vi "detect network devices.vi"(4 "remote timeout (300,000 ms)":u32=300000, 6 "detect all (F)":bool, 7 "local subnet only (F)":bool, 8 "error in":errorcluster, 10 "device class":T2, 11 "system session (localhost)":refnum<k21>="localhost") -> (0 "error out":errorcluster, 2 "devices":T1[](array[typedef]) {"product ID" format="%.0x"}, 3 "system session out":refnum<k21>)   [LabVIEW 2014, in "SMI.lvlib" / "Device.lvclass"]
uses:
  Device.lvclass
  device class selection.ctl
  network device information.ctl
  <vilib>/nisyscfg/Filter Mode.ctl
  <vilib>/nisyscfg/Close (Filter).vi
  <vilib>/nisyscfg/Close (Resources).vi
  <vilib>/regexp/Match Regular Expression.xnode
  <vilib>/nisyscfg/nisyscfg.lvlib
  <resource>/objmgr/niflexriosae.rc
  SMI.lvlib
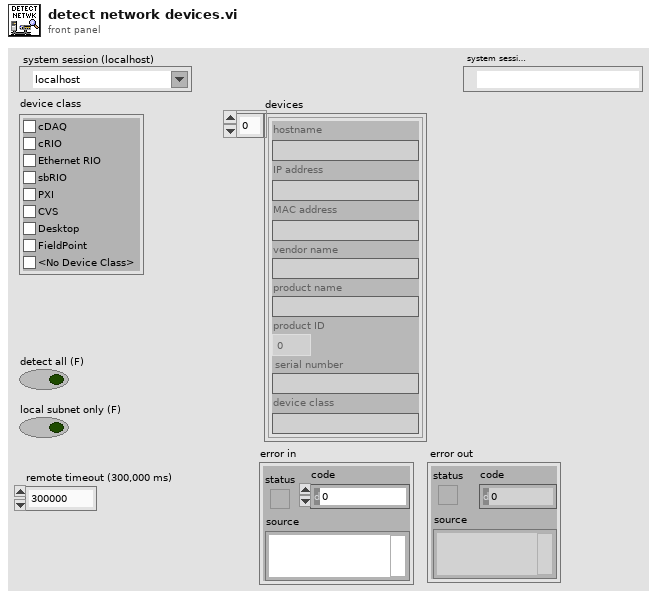
[diagram p1: front panel]
types:
  T1 = typedef "SMI.lvlib/Device.lvclass/network device information.ctl" = cluster{"hostname":string, "IP address":string, "MAC address":string, "vendor name":string, "product name":string, "product ID":u16, "serial number":string, "device class":string}
  T2 = typedef "SMI.lvlib/Device.lvclass/device class selection.ctl" = cluster{"cDAQ":bool, "cRIO":bool, "Ethernet RIO":bool, "sbRIO":bool, "PXI":bool, "CVS":bool, "Desktop":bool, "FieldPoint":bool, "<No Device Class>":bool}
  T3 = typedef "nisyscfg.lvlib/Filter Mode.ctl" = i32
  T4 = typedef "SMI.lvlib/Device.lvclass/device class.ctl" = enum16{"cDAQ", "cRIO", "Ethernet RIO", "sbRIO", "PXI", "CVS", "Desktop", "FieldPoint", "<No Device Class>", "<Detect All>"}
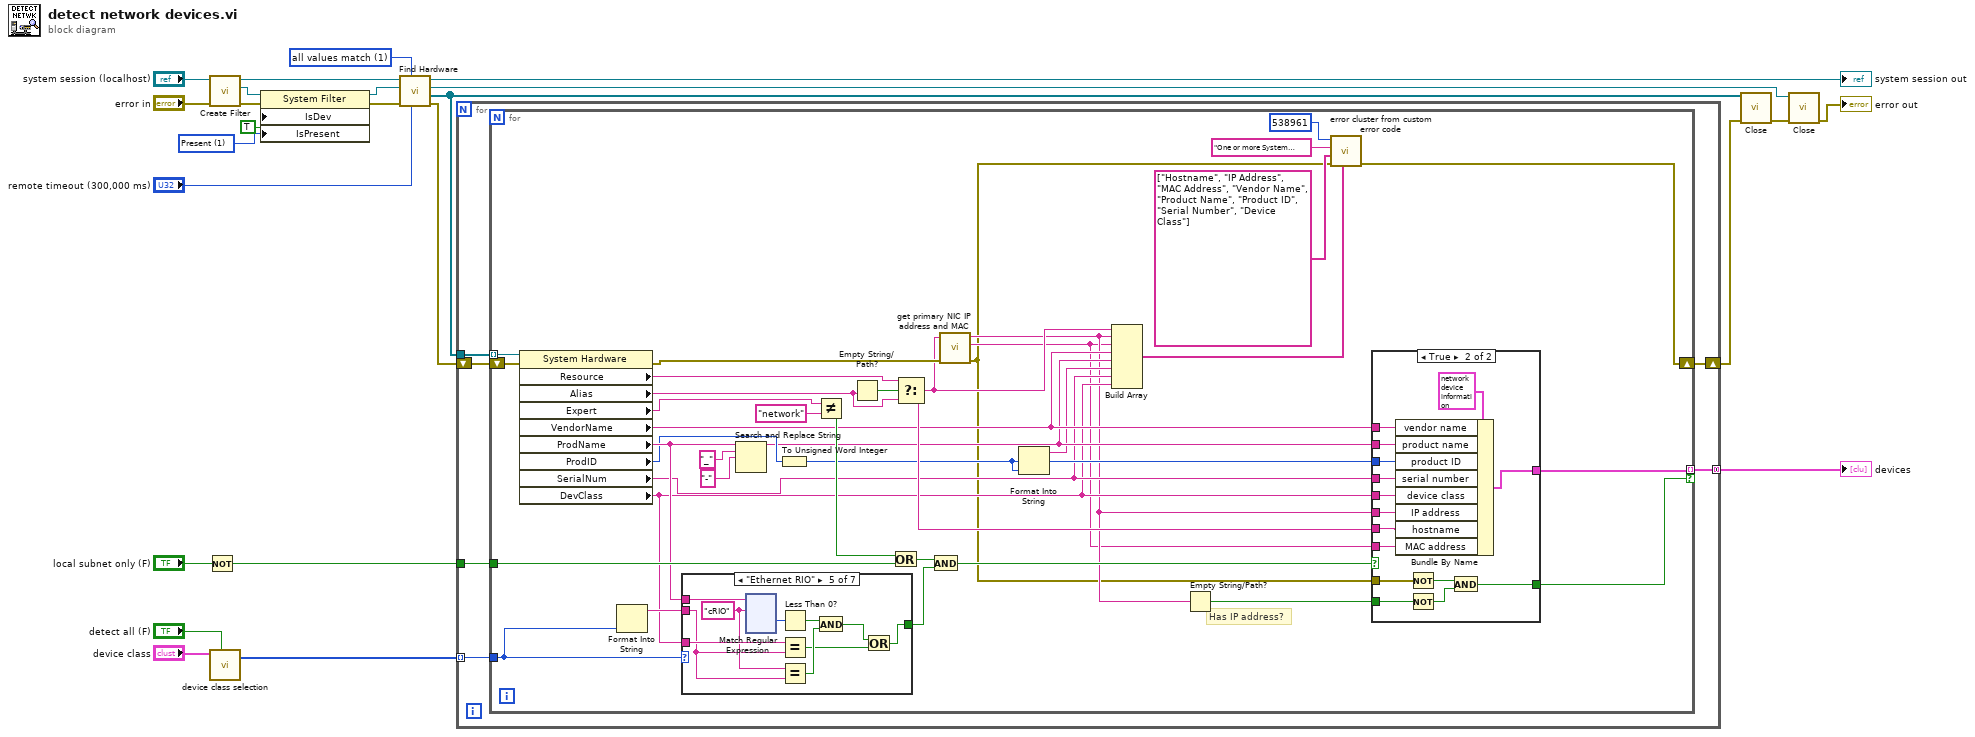
[diagram p0: block diagram]
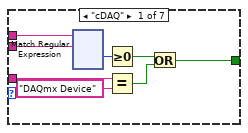
[diagram p3: hidden frame]
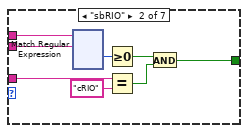
[diagram p4: hidden frame]
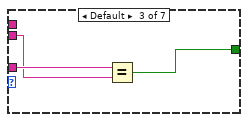
[diagram p5: hidden frame]
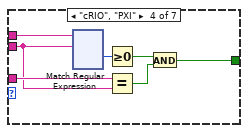
[diagram p6: hidden frame]
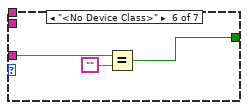
[diagram p7: hidden frame]
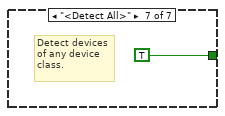
[diagram p8: hidden frame]
diagram:
  w4 = 1 items=["Initializing"=-2, "Unknown"=-1, "Not Present"=0, "Present"=1] ("Devices & Chassis:Is Present")
  w15 = T3 1 items=["all values match"=1, "any value matches"=2, "values do not match"=3, "all properties exist"=4] ("filter mode (all values match)")
  n1 = Not(x="local subnet only (F)") -> (.not. x?=w21:bool)
  n2 = call <vilib>:"Create Filter.vi"("error in (no error)"="error in", "Session in"="system session (localhost)") -> ("error out"=w20:errorcluster, "Filter out"=w19:refnum<k20>, "Session out"=w18:refnum<k21>)  [unwired: 7 in]
  n3 = call "device class selection.vi"("detect all (F)"="detect all (F)", "device classes"="device class") -> ("device class"=w1:T4[])  [unwired: 5 in]
  n4 = property class="System Filter"(reference=w19, error in=w20, "IsDev"=TRUE ("Is Chassis"), "IsPresent"=w4) -> (reference out=w16:refnum<k20>, error out=w17:errorcluster)
  n5 = call <vilib>:"Find Hardware.vi"("Remote Timeout (300,000 ms)"="remote timeout (300,000 ms)", "Filter Mode (all values match)"=w15, "error in (no error)"=w17, "Filter in"=w16, "Session in"=w18) -> ("error out"=w14:errorcluster, "Resources out"=w13:refnum<k20>[], "Filter out"=w11:refnum<k20>, "Session out"=→"system session out":refnum<k21>)  [unwired: 3 out]
  n6 = for {
    tunnel: w21 -> [w30]
    tunnel: w13 -> [w28]
    tunnel: w1 -> [w26] mode=indexing
    shift-right: [w27] -> w10
    shift-left: w14 -> [w29]
    tunnel: [w25] -> w3 mode=concatenating
    n7 = for {
      tunnel: w28 -> [w67] mode=indexing
      shift-right: [w34] -> w27
      shift-left: w29 -> [w66]
      tunnel: w30 -> [w65]
      tunnel: w26 -> [w49]
      tunnel: [w53] -> w25 mode=indexing if=w50
      # "Has IP address?"
      n8 = property class="System Hardware"(reference=w67, error in=w66) -> (error out=w43:errorcluster, "Resource"=w52:string, "Alias"=w64:string, "Expert"=w63:string, "VendorName"=w41:string, "ProdName"=w62:string, "ProdID"=w61:u32, "SerialNum"=w37:string, "DevClass"=w36:string)  [unwired: 1 out]
      n9 = Format Into String(w49) -> (resulting string=w48:string)  [unwired: 3 in, 1 out]
      n10 = case shown="\"Ethernet RIO\"" w49 {
        tunnel: w36 -> [w90 w212 w330 w336 w460 w578 _]
        tunnel: w62 -> [w91 w213 _ w337 w461 _ _]
        tunnel: [w86 w208 w329 w332 w452 w577 TRUE] -> w57
        tunnel: w48 -> [w84 w206 w328 w331 w457 _ _]
        frame "cDAQ" {
          n11 = xnode "Match Regular Expression"("input string"=w91, "regular expression"=w84) -> ("offset past match"=w89:i32)  [unwired: 4 in, 4 out]
          n12 = Greater Or Equal To 0?(x=w89) -> (x >= 0?=w87:bool)
          n13 = Equal?(x=w90, y="DAQmx Device") -> (x = y?=w88:bool)
          n14 = Or(x=w87, y=w88) -> (x .or. y?=w86:bool)
        }
        frame "sbRIO" {
          n15 = xnode "Match Regular Expression"("input string"=w213, "regular expression"=w206) -> ("offset past match"=w211:i32)  [unwired: 4 in, 4 out]
          n16 = Greater Or Equal To 0?(x=w211) -> (x >= 0?=w209:bool)
          n17 = Equal?(x=w212, y="cRIO") -> (x = y?=w210:bool)
          n18 = And(x=w209, y=w210) -> (x .and. y?=w208:bool)
        }
        frame Default {
          n19 = Equal?(x=w330, y=w328) -> (x = y?=w329:bool)
        }
        frame "cRIO", "PXI" {
          n20 = xnode "Match Regular Expression"("input string"=w337, "regular expression"=w331) -> ("offset past match"=w335:i32)  [unwired: 4 in, 4 out]
          n21 = Greater Or Equal To 0?(x=w335) -> (x >= 0?=w333:bool)
          n22 = Equal?(x=w336, y=w331) -> (x = y?=w334:bool)
          n23 = And(x=w333, y=w334) -> (x .and. y?=w332:bool)
        }
        frame "Ethernet RIO" {
          w458 = "cRIO" ("regular expression")
          n24 = xnode "Match Regular Expression"("input string"=w461, "regular expression"=w458) -> ("offset past match"=w459:i32)  [unwired: 4 in, 4 out]
          n25 = Less Than 0?(x=w459) -> (x < 0?=w456:bool)
          n26 = Equal?(x=w460, y=w457) -> (x = y?=w453:bool)
          n27 = Equal?(x=w458, y=w457) -> (x = y?=w455:bool)
          n28 = And(x=w456, y=w455) -> (x .and. y?=w454:bool)
          n29 = Or(x=w454, y=w453) -> (x .or. y?=w452:bool)
        }
        frame "<No Device Class>" {
          n30 = Equal?(x=w578, y="") -> (x = y?=w577:bool)
        }
        frame "<Detect All>" {
          # "Detect devices\nof any device\nclass."
        }
      }
      n31 = Search and Replace String(input string=w62, search string="_", replace string="-" ("replace string (\"\")")) -> (result string=w40:string)  [unwired: 5 in, 3 out]
      n32 = To Unsigned Word Integer(number=w61) -> (unsigned 16bit integer=w39:u16)
      n33 = Not Equal?(x=w63, y="network") -> (x != y?=w58:bool)
      n34 = Empty String/Path?(string/path=w64) -> (empty?=w60:bool)
      n35 = Or(x=w58, y=w65) -> (x .or. y?=w56:bool)
      n36 = Select(t=w52, s=w60, f=w64) -> (s? t:f=w42:string)
      n37 = And(x=w56, y=w57) -> (x .and. y?=w51:bool)
      n38 = call "get primary NIC IP address and MAC.vi"("error in"=w43, "system session"=w42) -> ("error out"=w31:errorcluster, "MAC address"=w32:string, "IP address"=w33:string)  [unwired: 7 in]
      n39 = Format Into String(w39) -> (resulting string=w38:string)  [unwired: 3 in, 1 out]
      n40 = Build Array(w42, w33, w32, w41, w40, w38, w37, w36) -> (w45:string[])
      n41 = Empty String/Path?(string/path=w33) -> (empty?=w35:bool)
      n42 = call "error cluster from custom error code.vi"("string values"=w45, "error in"=w31, "keys"=string[] ["Hostname", "IP Address", "MAC Address", "Vendor Name", "Product Name", "Product ID", "Serial Number", "Device Class"], "error message"="One or more System Hardware properties are not available for the network target.", "custom error code (0)"=538961 ("error code (0)")) -> ("error out"=w34:errorcluster)  [unwired: 6 in]
      n43 = case shown="True" w51 {
        selector: w51 -> [w68 _]
        tunnel: w41 -> [_ w83]
        tunnel: w36 -> [_ w82]
        tunnel: w37 -> [_ w81]
        tunnel: w40 -> [_ w79]
        tunnel: w39 -> [_ w78]
        tunnel: [_ w77] -> w53
        tunnel: w42 -> [_ w70]
        tunnel: [w68 w74] -> w50
        tunnel: w35 -> [_ w73]
        tunnel: w33 -> [_ w72]
        tunnel: w32 -> [_ w71]
        tunnel: w31 -> [_ w69]
        frame False {
        }
        frame True {
          n44 = Bundle By Name(cluster=T1 {"hostname"="cRIO-9014-Test", "IP address"="", "MAC address"="", "vendor name"="National Instruments", "product name"="", "product ID"=29071, "serial number"="00E86EAB", "device class"=""} ("Device Information"), "vendor name"=w83, "product name"=w79, "product ID"=w78, "serial number"=w81, "device class"=w82, "IP address"=w72, "hostname"=w70, "MAC address"=w71) -> (w77:T1)
          n45 = Not(x=w69) -> (.not. x?=w75:bool)
          n46 = Not(x=w73) -> (.not. x?=w76:bool)
          n47 = And(x=w75, y=w76) -> (x .and. y?=w74:bool)
        }
      }
    }
  }
  "devices" <- w3
  n48 = call-poly <vilib>:"Close.vi"("error in (no error)"=w10, "Resources in"=w13) -> ("error out"=w9:errorcluster)  [unwired: 9 in]
  n49 = call-poly <vilib>:"Close.vi"("error in (no error)"=w9, "Filter in"=w11) -> ("error out"=→"error out":errorcluster)  [unwired: 9 in]
